vi "RDC-Array-calc_propagation_const-formula.vi"(7 "dielectric":T1, 11 "Measured":T2) -> (2 "calc prop const":cdb[](array[numeric]))   [LabVIEW 2020, in "RDC-Reflection_Data_Computation.lvlib"]
doc: "Computes a propagation constant array per frequency of the Measured Common Format cluster from the properties of the selected coax dielectric (Teflon or Eccostock 0005), read with RDC-get_dielectric."
uses:
  RDC-Reflection_Data_Computation.lvlib
  Reflector/RFH-common_data_format.ctl
  RDC-dielectric_types.ctl
  Reflector/RFH-Reflection_File_Handler.lvlib
panel:
  out "alpha":dbl[](array[numeric])
  out "R'":dbl[](array[numeric])
  out "Rs":dbl[](array[numeric])
  out "alfa d":dbl[](array[numeric])
  out "beta":dbl[](array[numeric])
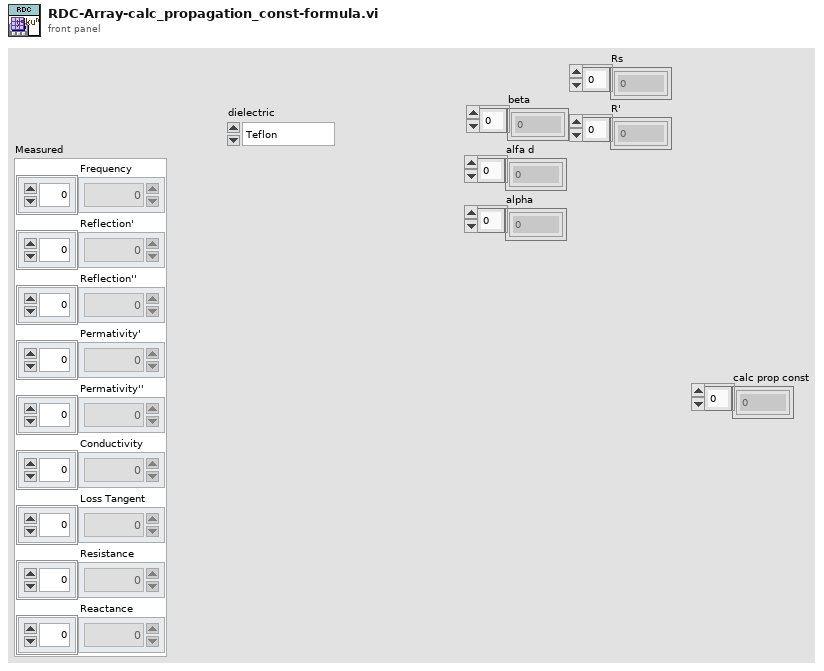
[diagram p1: front panel]
types:
  T1 = typedef "RDC-Reflection_Data_Computation.lvlib/RDC-dielectric_types.ctl" = enum16{"Teflon", "Eccostock 0005"}
  T2 = typedef "RFH-Reflection_File_Handler.lvlib/RFH-common_data_format.ctl" = cluster{"Frequency":dbl[], "Reflection'":dbl[], "Reflection''":dbl[], "Permativity'":dbl[], "Permativity''":dbl[], "Conductivity":dbl[], "Loss Tangent":dbl[], "Resistance":dbl[], "Reactance":dbl[]}
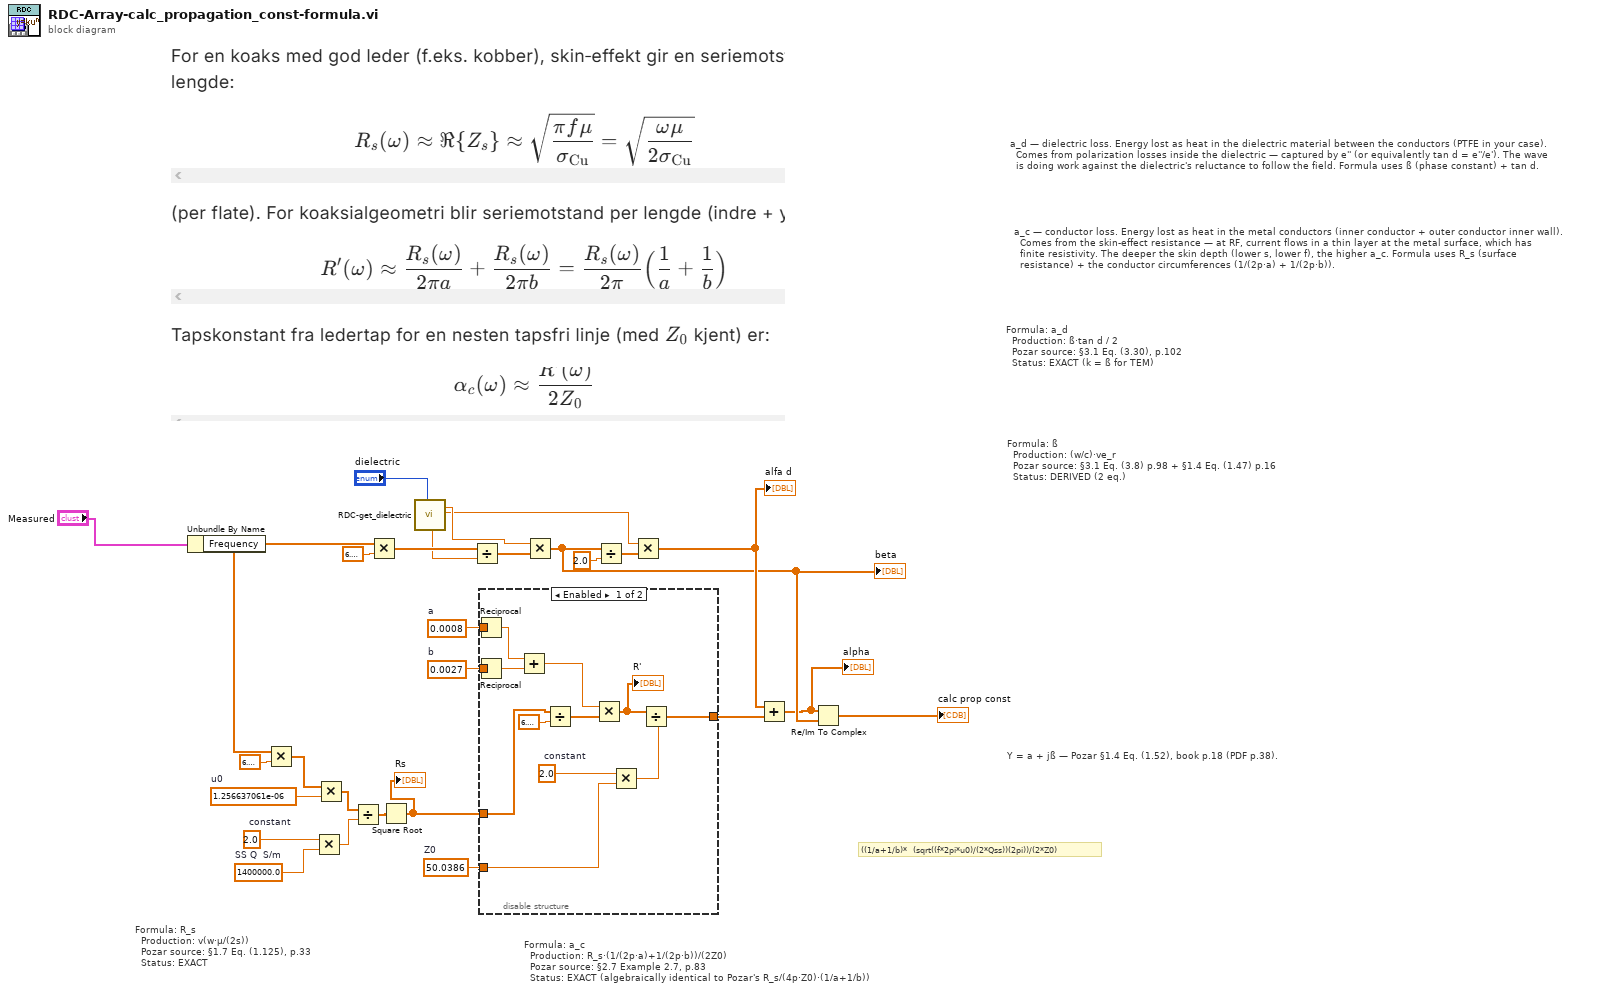
[diagram p0: block diagram]
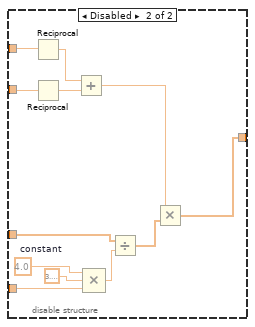
[diagram p2: hidden frame]
diagram:
  w8 = 50.0386  # Z0
  w10 = 0.0027  # b
  w11 = 0.0008  # a
  w18 = 2.0  # constant
  w14 = 1.256637061e-06  # u0
  w19 = 1400000.0  # SS Q  S/m
  # "Formula: R_s\n  Production: v(w·µ/(2s))\n  Pozar source: §1.7 Eq. (1.125), p.33\n  Status: EXACT"
  # "Formula: a_c\n  Production: R_s·(1/(2p·a)+1/(2p·b))/(2Z0)\n  Pozar source: §2.7 Example 2.7, p.83\n  Status: EXACT (algebraically identical to Pozar's R_s/(4p·Z0)·(1/a+1/b))"
  # "a_d — dielectric loss. Energy lost as heat in the dielectric material between the conductors (PTFE in your case).\n  Comes from polarization losses inside the dielectric — captured by e'' (or equivalently tan d = e''/e'). The wave\n  is doing work against the dielectric's reluctance to follow the field. Formula uses ß (phase constant) + tan d."
  # "a_c — conductor loss. Energy lost as heat in the metal conductors (inner conductor + outer conductor inner wall).\n  Comes from the skin-effect resistance — at RF, current flows in a thin layer at the metal surface, which has\n  finite resistivity. The deeper the skin depth (lower s, lower f), the higher a_c. Formula uses R_s (surface\n  resistance) + the conductor circumferences (1/(2p·a) + 1/(2p·b))."
  # "Formula: a_d\n  Production: ß·tan d / 2\n  Pozar source: §3.1 Eq. (3.30), p.102\n  Status: EXACT (k = ß for TEM)"
  # "Y = a + jß — Pozar §1.4 Eq. (1.52), book p.18 (PDF p.38)."
  # "Formula: ß\n  Production: (w/c)·ve_r\n  Pozar source: §3.1 Eq. (3.8) p.98 + §1.4 Eq. (1.47) p.16\n  Status: DERIVED (2 eq.)"
  # "((1/a+1/b)*  (sqrt((f*2pi*u0)/(2*Qss))(2pi))/(2*Z0)"
  n1 = Unbundle By Name("Measured") -> ("Frequency"=w6:dbl[])
  n2 = Multiply(x=w6, y=6.283185307179586) -> (x*y=w15:dbl[])
  n3 = Multiply(x=w18, y=w19) -> (x*y=w17:dbl)
  n4 = Multiply(x=w15, y=w14) -> (x*y=w13:dbl[])
  n5 = Divide(x=w13, y=w17) -> (x/y=w12:dbl[])
  n6 = Multiply(x=w6, y=6.283185307179586) -> (x*y=w27:dbl[])
  n7 = Square Root(x=w12) -> (sqrt(x)=w9:dbl[])
  "Rs" <- w9
  n8 = call "RDC-get_dielectric.vi"("dielectric"="dielectric") -> ("speed of light C"=w26:dbl, "sqrt(er)"=w24:dbl, "tanQ"=w21:dbl)  [unwired: 13 in, 3 out]
  n9 = Divide(x=w27, y=w26) -> (x/y=w25:dbl[])
  n10 = disable-structure shown="Enabled" {
    disable-tunnel: w11 -> [w41 w46]
    disable-tunnel: w10 -> [w40 w45]
    disable-tunnel: w9 -> [w37 w53]
    disable-tunnel: w8 -> [w31 w52]
    disable-tunnel: [w29 w42] -> w7
    frame Enabled {
      w32 = 2.0  # constant
      n11 = Reciprocal(x=w41) -> (1/x=w39:dbl)
      n12 = Reciprocal(x=w40) -> (1/x=w38:dbl)
      n13 = Add(x=w39, y=w38) -> (x+y=w34:dbl)
      n14 = Divide(x=w37, y=6.283185307179586) -> (x/y=w35:dbl[])
      n15 = Multiply(x=w34, y=w35) -> (x*y=w33:dbl[])
      "R'" <- w33
      n16 = Multiply(x=w32, y=w31) -> (x*y=w30:dbl)
      n17 = Divide(x=w33, y=w30) -> (x/y=w29:dbl[])
    }
    frame Disabled {
      w51 = 4.0  # constant
      n18 = Reciprocal(x=w46) -> (1/x=w48:dbl)
      n19 = Reciprocal(x=w45) -> (1/x=w47:dbl)
      n20 = Add(x=w48, y=w47) -> (x+y=w43:dbl)
      n21 = Compound Arithmetic op=MULTIPLY(w51, 3.141592653589793, w52) -> (w49:dbl)
      n22 = Divide(x=w53, y=w49) -> (x/y=w44:dbl[])
      n23 = Multiply(x=w43, y=w44) -> (x*y=w42:dbl[])
    }
  }
  n24 = Multiply(x=w24, y=w25) -> (x*y=w2:dbl[])
  "beta" <- w2
  n25 = Divide(x=w2, y=2.0 ("value")) -> (x/y=w22:dbl[])
  n26 = Multiply(x=w21, y=w22) -> (x*y=w20:dbl[])
  "alfa d" <- w20
  n27 = Add(x=w20, y=w7) -> (x+y=w1:dbl[])
  "alpha" <- w1
  n28 = Re/Im To Complex(1:w2, 2:w1) -> (0:→"calc prop const":cdb[])
